vi "Save CSV (Async).vi"(5 "CSV File Ref":refnum<vi>, 7 "MONITOR TABLE Ref":refnum<vi>, 8 "error in (no error)":errorcluster, 11 "Measurement UI Queue":refnum<queue>) -> (0 "error out":errorcluster)   [LabVIEW 2025, in "I2C Bus Monitor UI.lvlib"]
uses:
  I2C Bus Monitor UI.lvlib
  Save CSV.vi
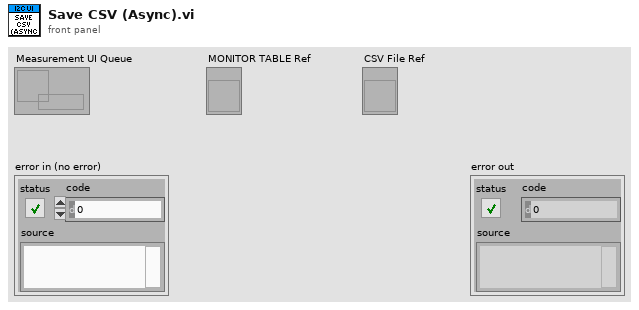
[diagram p1: front panel]
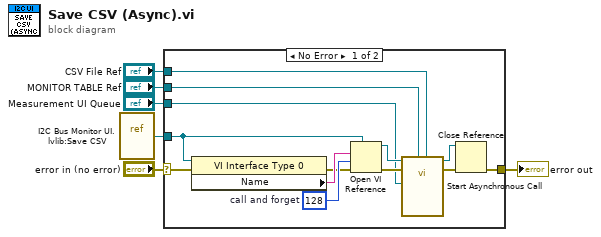
[diagram p0: block diagram]
diagram:
  n1 = vi-ref "I2C Bus Monitor UI.lvlib:Save CSV.vi"() -> (w6:refnum<vi>)
  n2 = case shown="No Error" "error in (no error)" {
    selector: "error in (no error)" -> [w11 w20]
    tunnel: w6 -> [w12 _]
    tunnel: [w10 w20] -> w4
    tunnel: "CSV File Ref" -> [w9 _]
    tunnel: "MONITOR TABLE Ref" -> [w8 _]
    tunnel: "Measurement UI Queue" -> [w7 _]
    frame No Error {
      w19 = 128  # call and forget
      n3 = property class="VI Interface Type 0"(reference=w12, error in=w11) -> (error out=w13:errorcluster, "Name"=w14:string)  [unwired: 1 out]
      n4 = Open VI Reference(type specifier VI Refnum (for type only)=w12, vi path=w14, options=w19, error in (no error)=w13) -> (vi reference=w18:refnum<vi>, error out=w17:errorcluster)  [unwired: 2 in]
      n5 = call-by-ref "Start Asynchronous Call"(reference=w18, error in=w17, "CSV FILE PATH Ref"=w9, "MONITOR TABLE Ref"=w8, "Measurement UI Queue"=w7) -> (reference out=w15:refnum<vi>, error out=w16:errorcluster)  [unwired: 8 in, 1 out]
      n6 = Close Reference(reference=w15, error in (no error)=w16) -> (error out=w10:errorcluster)
    }
    frame Error {
    }
  }
  "error out" <- w4
